vi "onTestDiscovery.vi"(8 "error in (no error)":errorcluster, 11 "Test Runner.Library in":refnum<class "Test Runner.Library.lvclass">) -> (0 "error out":errorcluster, 2 "Tests VIs":path[](array[path]), 3 "Test Runner.Library out":refnum<class "Test Runner.Library.lvclass">)   [LabVIEW 2020, in "Caraya.lvlib" / "Test Runner.Library.lvclass"]
uses:
  Test Runner.Library.lvclass
  C:/projects/caraya/src/classes/Test Runner/Test Runner.lvclass
  Test Runner.Library.lvclass/Test Runner.Library.ctl
  Test Runner/Test Runner.lvclass/Test Runner.ctl
  Test Runner/Test Runner.lvclass
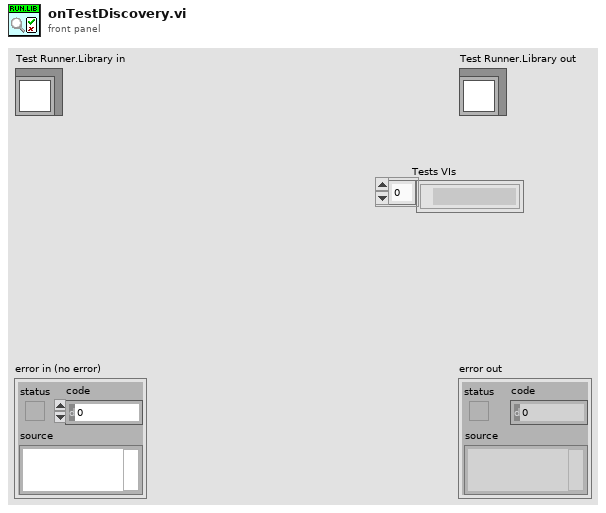
[diagram p1: front panel]
types:
  T1 = typedef "NI_FileType.lvlib/LVFileType.ctl" = enum32{"Invalid file", "Unknown type", "Instrument", "Control", "Polymorphic VI", "Project", "Library", "LVClass", "XControl", "XNode", "Shared library", ".NET assembly", "ActiveX interface", "CIN", "Run-time menu", "Palette menu", "Help file", "LLB", "XNode Edit Dependency", "Class Private Data Control", "Statechart", "MathScript .m file", "Ladder Diagram", "LVLibp", "XNode Build Dependency"}
  T2 = cluster{"path":path, "delimited name":string, "type":T1, "iState":u32, "iStyle":u16, "wStyle":u16, "buttons":u16, "viflags":u32, "viflags2":u32, "links":u32[]}[]
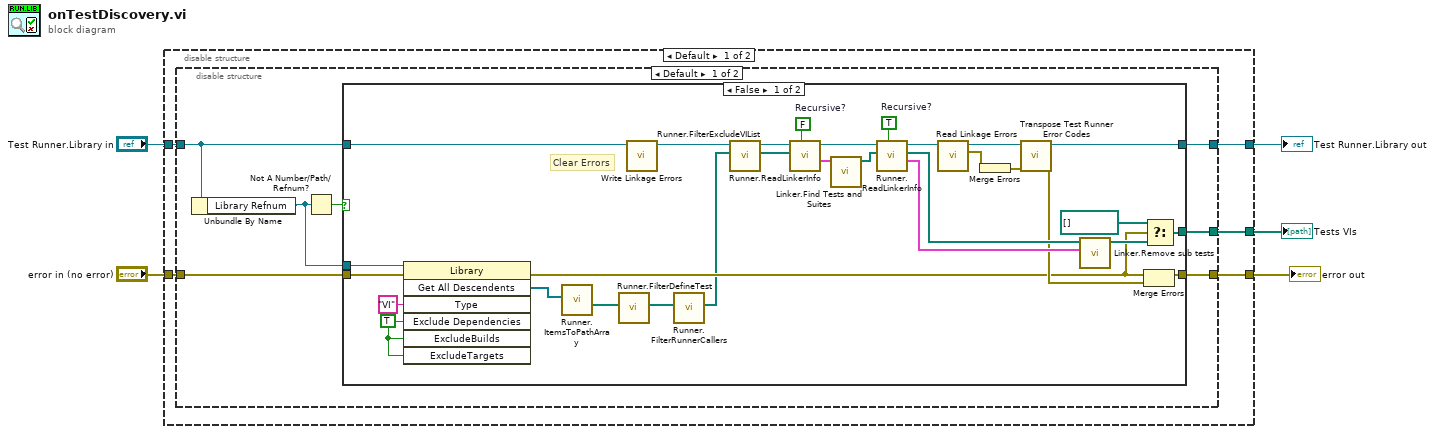
[diagram p0: block diagram]
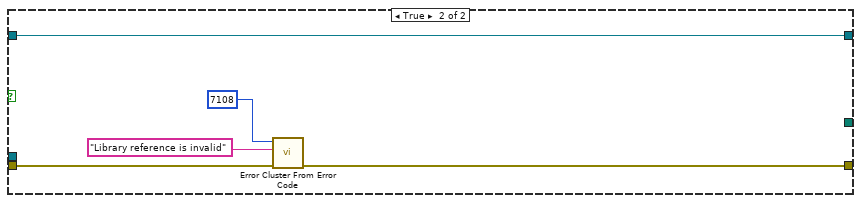
[diagram p2: hidden frame]
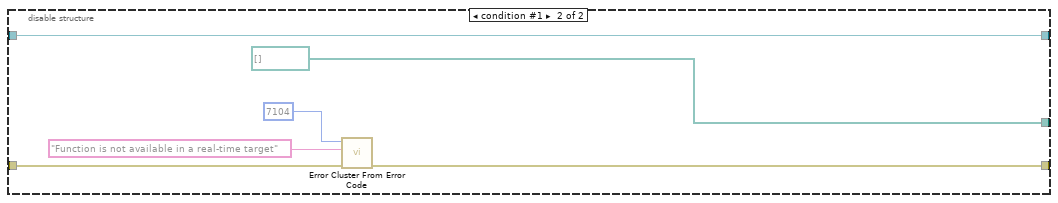
[diagram p3: hidden frame]
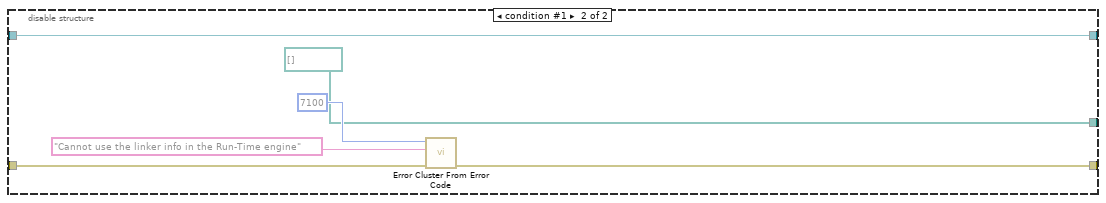
[diagram p4: hidden frame]
diagram:
  n1 = disable-structure shown="Default" {
    disable-tunnel: [w10 w62] -> w3
    disable-tunnel: "Test Runner.Library in" -> [w6 w61]
    disable-tunnel: [w9 w61] -> w1
    disable-tunnel: [w8 path[] [] ("Test VIs")] -> w2
    disable-tunnel: "error in (no error)" -> [w7 w59]
    frame condition #0 (active) {
      n2 = disable-structure shown="Default" {
        disable-tunnel: [w17 w54] -> w10
        disable-tunnel: [w16 w58] -> w9
        disable-tunnel: [w15 path[] [] ("Test VIs")] -> w8
        disable-tunnel: w7 -> [w13 w55]
        disable-tunnel: w6 -> [w12 w58]
        frame condition #0 (active) {
          n3 = Unbundle By Name(w12) -> ("Library Refnum"=w11:refnum<vi>)
          n4 = Not A Number/Path/Refnum?(number/path/refnum=w11) -> (NaN/Path/Refnum?=w14:bool)
          n5 = case shown="False" w14 {
            tunnel: [w26 w48] -> w17
            tunnel: [w47 _] -> w15
            tunnel: w11 -> [w41 _]
            tunnel: w12 -> [w37 w52]
            tunnel: [w23 w52] -> w16
            tunnel: w13 -> [w42 w49]
            frame False {
              w36 = FALSE  # Recursive?
              w35 = TRUE  # Recursive?
              w45 = TRUE ("ExcludeDependencies")
              # "Clear Errors"
              n6 = invoke class="Library" method="Get All Descendents"(reference=w41, error in=w42, "Type"="VI", "Exclude Dependencies"=w45, "ExcludeBuilds"=w45, "ExcludeTargets"=w45) -> (error out=w25:errorcluster, "All Descendents"=w40:refnum<vi>[])  [unwired: 1 in, 5 out]
              n7 = call "Runner.ItemsToPathArray.vi"("Project Items"=w40) -> ("Paths"=w39:path[])  [unwired: 10 in]
              n8 = call "Runner.FilterDefineTest.vi"("Paths"=w39) -> ("Filtered Paths"=w38:path[])  [unwired: 10 in]
              n9 = call "Write Linkage Errors.vi"("Test Runner in"=w37) -> ("Test Runner out"=w20:refnum<class "Test Runner.Library.lvclass">)  [unwired: 9 in, 1 out]
              n10 = call "Runner.FilterRunnerCallers.vi"("Paths"=w38) -> ("Filtered Paths"=w19:path[])  [unwired: 10 in]
              n11 = call "Runner.FilterExcludeVIList.vi"("Paths"=w19, "Test Runner"=w20) -> ("Filtered Paths"=w18:path[], "Test Runner"=w21:refnum<class "Test Runner.Library.lvclass">)  [unwired: 8 in]
              n12 = call "Runner.ReadLinkerInfo.vi"("Recursive?"=w36, "VI Paths"=w18, "Test Runner in"=w21) -> ("Linker:Read Info From File"=w33:T2, "Test Runner out"=w34:refnum<class "Test Runner.Library.lvclass">)  [unwired: 5 in, 2 out]
              n13 = call "Linker.Find Tests and Suites.vi"("Linker:Read Info From File"=w33) -> ("All VIs defining a test (excluding those defining a suite)"=w32:path[])  [unwired: 8 in, 2 out]
              n14 = call "Runner.ReadLinkerInfo.vi"("Recursive?"=w35, "VI Paths"=w32, "Test Runner in"=w34) -> ("Linker:Read Info From File"=w30:T2, "VI Paths (dup)"=w31:path[], "Test Runner out"=w24:refnum<class "Test Runner.Library.lvclass">)  [unwired: 5 in, 1 out]
              n15 = call "Read Linkage Errors.vi"("Test Runner in"=w24) -> ("Linkage Errors"=w22:errorcluster[], "Test Runner out"=w28:refnum<class "Test Runner.Library.lvclass">)  [unwired: 8 in, 1 out]
              n16 = Merge Errors(w22) -> (w29:errorcluster)
              n17 = call-dynamic "Transpose Test Runner Error Codes.vi"("error in (no error)"=w29, "Test Runner in"=w28) -> ("error out"=w27:errorcluster, "Test Runner out"=w23:refnum<class "Test Runner.Library.lvclass">)  [unwired: 8 in]
              n18 = call "Linker.Remove sub tests.vi"("Linker.Read Info From File"=w30, "Tests"=w31) -> ("Array"=w43:path[])  [unwired: 9 in]
              n19 = Merge Errors(w25, w27) -> (w26:errorcluster)
              n20 = Select(t=path[] [], s=w25, f=w43) -> (s? t:f=w47:path[])
            }
            frame True {
              n21 = call <vilib>:"Error Cluster From Error Code.vi"("error in (no error)"=w49, "error message (\"\")"="Library reference is invalid" ("error message (\"\")"), "error code (0)"=7108) -> ("error out"=w48:errorcluster)  [unwired: 6 in]
            }
          }
        }
        frame condition #1 {
          n22 = call <vilib>:"Error Cluster From Error Code.vi"("error in (no error)"=w55, "error message (\"\")"="Function is not available in a real-time target" ("error message (\"\")"), "error code (0)"=7104) -> ("error out"=w54:errorcluster)  [unwired: 6 in]
        }
      }
    }
    frame condition #1 {
      n23 = call <vilib>:"Error Cluster From Error Code.vi"("error in (no error)"=w59, "error message (\"\")"="Cannot use the linker info in the Run-Time engine" ("error message (\"\")"), "error code (0)"=7100) -> ("error out"=w62:errorcluster)  [unwired: 6 in]
    }
  }
  "error out" <- w3
  "Test Runner.Library out" <- w1
  "Tests VIs" <- w2
